vi "tcpip_forward.vi"() -> ()   [LabVIEW 2017]
doc: "Ilustrates how to establish an TCP/IP tunnel through an SSH server."
uses:
  <vilib>/Utility/error.llb/DialogType.ctl
  libssh2/libssh2_session_handshake_tcp.vi
  libssh2/libssh2_init_default.vi
  libssh2/libssh2_session_init_ex.vi
  <vilib>/Utility/tcp.llb/TCP Get Raw Net Object.vi
  libssh2/libssh2_session_handshake_socket.vi
  libssh2/libssh2_userauth_password_ex.vi
  libssh2/libssh2_channel_forward_listen_ex.vi
  libssh2/libssh2_channel_write_ex.vi
  libssh2/libssh2_channel_read_ex.vi
  libssh2/libssh2_session_disconnect_ex.vi
  libssh2/libssh2.lvlib
panel:
  out "bound_port":i32
  in  "stop":bool
  in  "local_destport":i32=4444
  in  "local_destip":string="localhost"
  in  "wantport":i32=2222
  in  "server_ip":string="127.0.0.1"
  in  "password":string
  in  "username":string
  out "error out":errorcluster
  # "SSH server connection"
  # "This is the port that the SSH server should be listening on.\nThe server may choose a different port, indicated by bound_port."
  # "This is the hostname and port to forward the TCP\nconnection to.\n\nAll data received from the SSH server is forwarded\nto this endpoint."
  # "1) Configure your settings\n2) Run this VI\n3) Open a TCP/IP listener for local_destip and local_destport\n4) Open a TCP/IP connection to remote_listenhost and bound_port\n \nNOTE:\nIf you can't establish a connection then your SSH server's firewall may\nblock the port. In this case you can try opening a TCP/IP connection\nfrom the SSH server itself (connect to itself on the bound port).\nFor example, using \"netcat <remote_listenhost> <bound_port>\"\n\n5) Send some data => You should see the incomming data on your TCP listener\n6) Press STOP to close the tunnel"
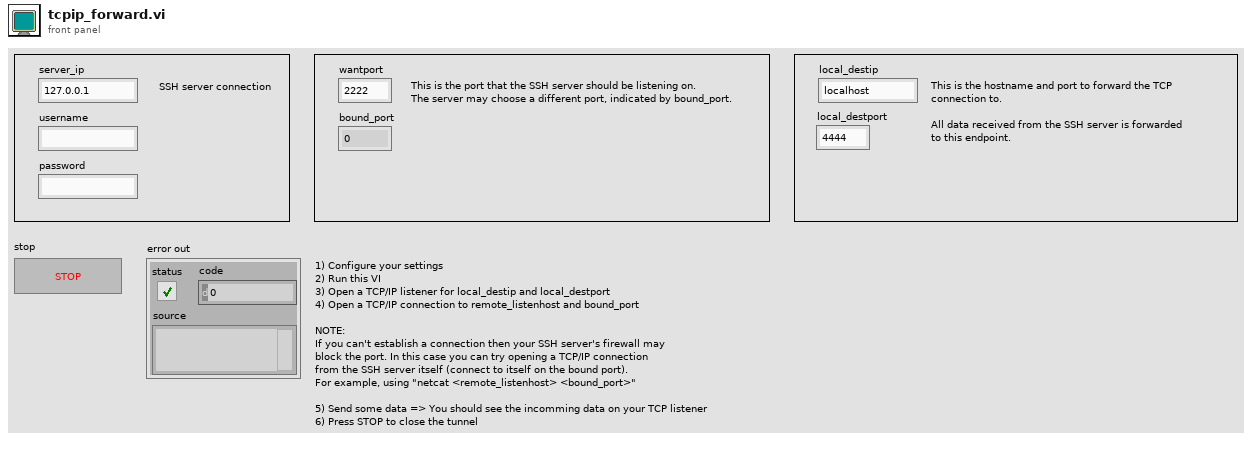
[diagram p1: front panel]
types:
  T1 = typedef "libssh2.lvlib/Session Refnum.ctl" = refnum<k1>
  T2 = typedef "libssh2.lvlib/Listener Refnum.ctl" = refnum<k1>
  T3 = typedef "libssh2.lvlib/Channel Refnum.ctl" = refnum<k1>
  T4 = enum16{"Standard", "Buffered", "CRLF", "Immediate"}
  T5 = typedef "DialogType.ctl" = u16
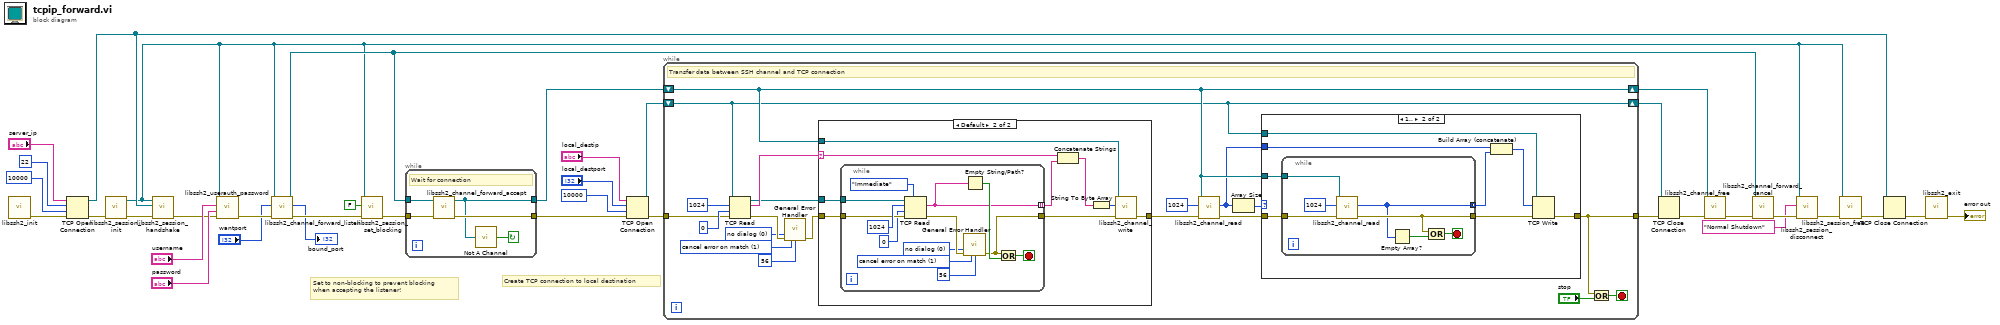
[diagram p0: block diagram]
diagram:
  # "Create TCP connection to local destination"
  # "Set to non-blocking to prevent blocking\nwhen accepting the listener!"
  n1 = call-poly "libssh2_init.vi"() -> ("error out"=w33:errorcluster)  [unwired: 11 in]
  n2 = TCP Open Connection(address="server_ip", remote port or service name=u16 22, timeout ms (60000)=10000, error in (no error)=w33) -> (connection ID=w6:refnum<k5>, error out=w7:errorcluster)  [unwired: 1 in]
  n3 = call "libssh2_session_init.vi"("error in (no error)"=w7) -> ("error out"=w32:errorcluster, "session"=w3:T1)  [unwired: 9 in]
  n4 = call-poly "libssh2_session_handshake.vi"("error in (no error)"=w32, "tcp connection"=w6, "session"=w3) -> ("error out"=w13:errorcluster)  [unwired: 8 in]
  n5 = call "libssh2_userauth_password.vi"("error in (no error)"=w13, "password"="password", "username"="username", "session"=w3) -> ("error out"=w30:errorcluster)  [unwired: 7 in]
  n6 = call "libssh2_channel_forward_listen.vi"("error in (no error)"=w30, "port in"="wantport", "session"=w3) -> ("error out"=w28:errorcluster, "port out"=→"bound_port":i32, "listener"=w23:T2)  [unwired: 6 in]
  n7 = call "libssh2_session_set_blocking.vi"("error in (no error)"=w28, "blocking"=FALSE, "session"=w3) -> ("error out"=w5:errorcluster)  [unwired: 8 in]
  n8 = while {
    tunnel: [w39] -> w27
    tunnel: w23 -> [w41]
    tunnel: [w38] -> w10
    tunnel: w5 -> [w40]
    stop <- w37 continue-if-true
    # "Wait for connection"
    n9 = call "libssh2_channel_forward_accept.vi"("error in (no error)"=w40, "listener"=w41) -> ("error out"=w39:errorcluster, "channel"=w38:T3)  [unwired: 8 in]
    n10 = call "Not A Channel.vi"("channel"=w38) -> ("Not a Channel?"=w37:bool)
  }
  n11 = TCP Open Connection(address="local_destip", remote port or service name="local_destport", timeout ms (60000)=10000, error in (no error)=w27) -> (connection ID=w9:refnum<k5>, error out=w2:errorcluster)  [unwired: 1 in]
  n12 = while {
    tunnel: w2 -> [w52]
    tunnel: [w48] -> w8
    shift-right: [w54] -> w12
    shift-left: w10 -> [w54]
    shift-right: [w49] -> w11
    shift-left: w9 -> [w49]
    stop <- w46 stop-if-true
    w43 = T5 0 items=["no dialog", "OK message", "continue or stop message", "OK message + warnings", "continue/stop + warnings"] ("type of dialog (OK msg:1)")
    w45 = 1 items=["no exception", "cancel error on match", "set error on match"] ("[exception action] (none:0)")
    # "Transfer data between SSH channel and TCP connection"
    n13 = TCP Read(connection ID=w49, bytes to read=1024, error in (no error)=w52, 9:0 ("timeout ms (25000)")) -> (connection ID out=w50:refnum<k5>, data out=w60:string, error out=w53:errorcluster)  [unwired: 1 in]
    n14 = call <vilib>:"General Error Handler.vi"("type of dialog (OK msg:1)"=w43, "error in (no error)"=w53, "[exception action] (none:0)"=w45, "[exception code]"=56 ("specific error code to clear (0: all)")) -> ("error out"=w51:errorcluster)  [unwired: 7 in, 4 out]
    n15 = case shown="Default" w60 {
      selector: w60 -> [_ w81]
      tunnel: [w78 w84] -> w56
      tunnel: w50 -> [_ w87]
      tunnel: w51 -> [w78 w86]
      tunnel: w54 -> [_ w83]
      frame "" {
      }
      frame Default {
        n16 = while {
          tunnel: [w92] -> w85
          tunnel: w87 -> [w98]
          tunnel: w86 -> [w95]
          tunnel: [w91] -> w82 mode=indexing
          stop <- w96 stop-if-true
          w88 = T5 0 items=["no dialog", "OK message", "continue or stop message", "OK message + warnings", "continue/stop + warnings"] ("type of dialog (OK msg:1)")
          w89 = 1 items=["no exception", "cancel error on match", "set error on match"] ("[exception action] (none:0)")
          n17 = TCP Read(connection ID=w98, bytes to read=1024, error in (no error)=w95, 7:T4."Immediate" ("mode (standard)"), 9:0 ("timeout ms (25000)")) -> (data out=w91:string, error out=w93:errorcluster)  [unwired: 1 out]
          n18 = call <vilib>:"General Error Handler.vi"("type of dialog (OK msg:1)"=w88, "error in (no error)"=w93, "[exception action] (none:0)"=w89, "[exception code]"=56 ("specific error code to clear (0: all)")) -> ("error out"=w92:errorcluster)  [unwired: 7 in, 4 out]
          n19 = Empty String/Path?(string/path=w91) -> (empty?=w97:bool)
          n20 = Or(x=w92, y=w97) -> (x .or. y?=w96:bool)
        }
        n21 = Concatenate Strings(w81, w82) -> (w80:string)
        n22 = String To Byte Array(string=w80) -> (unsigned byte array=w79:u8[])
        n23 = call "libssh2_channel_write.vi"("error in (no error)"=w85, "buffer"=w79, "channel"=w83) -> ("error out"=w84:errorcluster)  [unwired: 7 in, 1 out]
      }
    }
    n24 = call "libssh2_channel_read.vi"("error in (no error)"=w56, "buffer length"=1024 ("buflen"), "channel"=w54) -> ("error out"=w55:errorcluster, "buffer"=w42:u8[])  [unwired: 7 in]
    n25 = Array Size(array=w42) -> (size(s)=w58:i32)
    n26 = case shown="1.." w58 {
      tunnel: [w62 w68] -> w48
      tunnel: w54 -> [_ w70]
      tunnel: w49 -> [_ w67]
      tunnel: w55 -> [w62 w69]
      tunnel: w42 -> [_ w66]
      frame Default {
      }
      frame 1.. {
        n27 = while {
          tunnel: w70 -> [w73]
          tunnel: w69 -> [w74]
          tunnel: [w71] -> w65 mode=concatenating
          tunnel: [w72] -> w63
          stop <- w77 stop-if-true
          n28 = call "libssh2_channel_read.vi"("error in (no error)"=w74, "buffer length"=1024 ("buflen"), "channel"=w73) -> ("error out"=w72:errorcluster, "buffer"=w71:u8[])  [unwired: 7 in]
          n29 = Empty Array?(array=w71) -> (empty?=w76:bool)
          n30 = Compound Arithmetic op=OR(w72, w76) -> (w77:bool)
        }
        n31 = Build Array (concatenate)(w66, w65) -> (w64:u8[])
        n32 = TCP Write(connection ID=w67, data in=w64, error in (no error)=w63) -> (error out=w68:errorcluster)  [unwired: 1 in, 2 out]
      }
    }
    n33 = Or(x=w48, y="stop") -> (x .or. y?=w46:bool)
  }
  n34 = TCP Close Connection(connection ID=w11, error in (no error)=w8) -> (error out=w21:errorcluster)  [unwired: 1 in, 1 out]
  n35 = call "libssh2_channel_free.vi"("error in (no error)"=w21, "channel"=w12) -> ("error out"=w24:errorcluster)  [unwired: 9 in]
  n36 = call "libssh2_channel_forward_cancel.vi"("error in (no error)"=w24, "listener"=w23) -> ("error out"=w22:errorcluster)  [unwired: 9 in]
  n37 = call "libssh2_session_disconnect.vi"("error in (no error)"=w22, "description"="Normal Shutdown", "session"=w3) -> ("error out"=w31:errorcluster)  [unwired: 8 in]
  n38 = call "libssh2_session_free.vi"("error in (no error)"=w31, "session"=w3) -> ("error out"=w14:errorcluster)  [unwired: 9 in]
  n39 = TCP Close Connection(connection ID=w6, error in (no error)=w14) -> (error out=w16:errorcluster)  [unwired: 1 in, 1 out]
  n40 = call "libssh2_exit.vi"("error in (no error)"=w16) -> ("error out"=→"error out":errorcluster)  [unwired: 10 in]
